vi "Measurement Logic.vi"() -> ()   [LabVIEW 2021, in "Load Transient Response_PMIC.lvlib"]
uses:
  Load Transient Response_PMIC.lvlib
  Measurement Configuration.ctl
  Measurement Results.ctl
  <vilib>/Plug-In SDKs/Measurements/Measure Call Context/Measure Call Context.lvclass
  <instrlib>/niDCPower/nidcpower.llb/niDCPower Sense.ctl
  <instrlib>/niDCPower/nidcpower.llb/niDCPower Source Mode.ctl
  <instrlib>/niDCPower/nidcpower.llb/niDCPower Wait For Event - Event.ctl
  <instrlib>/niDCPower/nidcpower.llb/niDCPower Output Function.ctl
  <instrlib>/niDCPower/nidcpower.llb/niDCPower Aperture Time Units.ctl
  <instrlib>/niDCPower/nidcpower.llb/niDCPower Configure Digital Edge Measure Trigger With Channels.vi
panel:
  out "measure call context out":refnum<class "Measure Call Context.lvclass">
  in  "measure call context in":refnum<class "Measure Call Context.lvclass">
  out "measurement results":T1
  in  "measurement configuration":T2={"Mode of operation"=enum."Perform measurement", "DUT setup time"=1.0, "Nominal output voltage"=3.3, "Source resource name"="", "Source sense"=1009, "Source current limit"=25.0, "Source voltage level"=12.0, "Source transient response"=1041, "Source voltage gain bandwidth"=2000.0, "Source voltage compensation frequency"=3530.0, "Source voltage pole-zero ratio"=2.0, "Load resource name"="", "Load sense"=1009, "Load voltage limit range"=6.0, "Load current level range"=6.0, "Load sample rate"=1800000.0, "Load current set point 1"=1.0, "Load current set point 2"=22.0, "Load current delay t1"=0.001, "Load current pulse duration"=0.001, "Load current delay t2"=0.001, "Load current rising slew rate"=24.0, "Load current falling slew rate"=24.0, "Load transient response"=3, "Load current gain bandwidth"=14000.0, "Load current compensation frequency"=180000.0, "Load current pole-zero ratio"=0.3} {"Load transient response" items=["Slow"=1041, "Normal"=1038, "Fast"=1039, "Custom"=1042]; "Load current rising slew rate" format="%#_6p"; "Load sense" items=["Local"=1008, "Remote"=1009]; "Source transient response" items=["Slow"=1041, "Normal"=1038, "Fast"=1039, "Custom"=1042]; "Source sense" items=["Local"=1008, "Remote"=1009]; "Nominal output voltage" format="%#_6p"}
  out "error out":errorcluster
  in  "error in":errorcluster
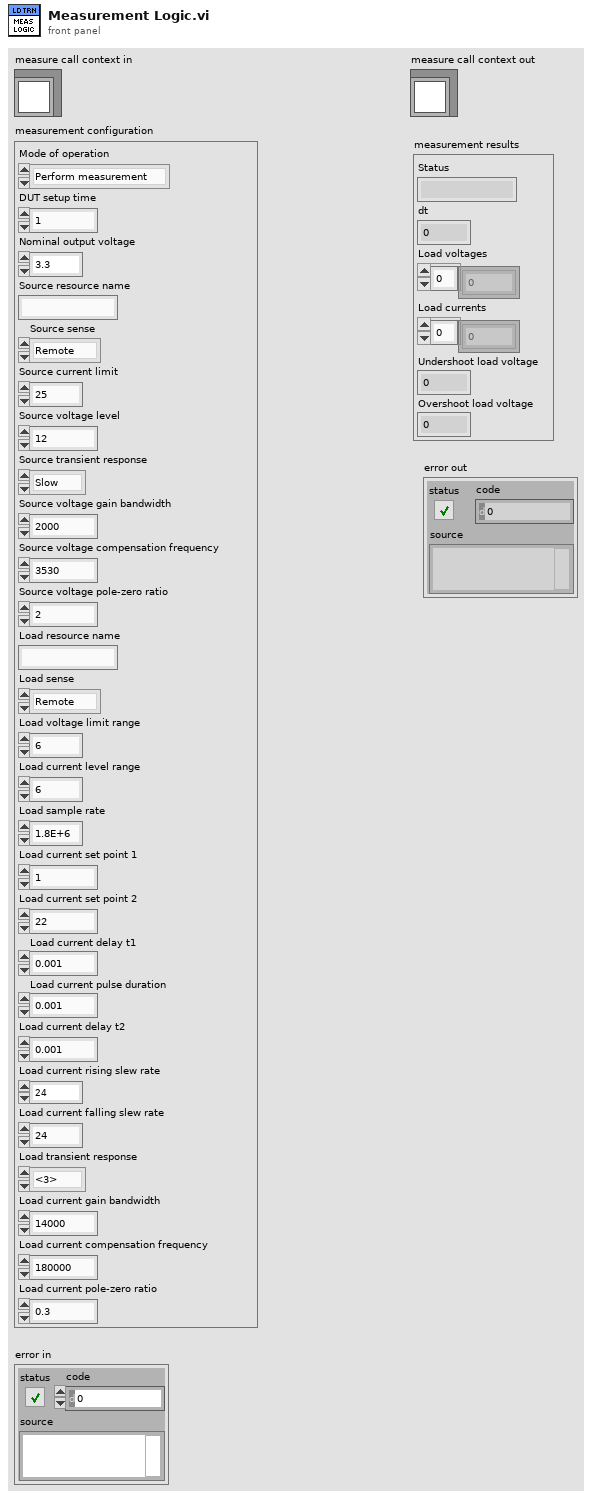
[diagram p1: front panel]
types:
  T1 = typedef "Load Transient Response_PMIC.lvlib/Measurement Results.ctl" = cluster{"Status":string, "dt":dbl, "Load voltages":dbl[], "Load currents":dbl[], "Undershoot load voltage":dbl, "Overshoot load voltage":dbl}
  T2 = typedef "Load Transient Response_PMIC.lvlib/Measurement Configuration.ctl" = cluster{"Mode of operation":enum32{"Power on the DUT", "Perform measurement", "Power off the DUT"}, "DUT setup time":dbl, "Nominal output voltage":dbl, "Source resource name":string, "Source sense":i32, "Source current limit":dbl, "Source voltage level":dbl, "Source transient response":i32, "Source voltage gain bandwidth":dbl, "Source voltage compensation frequency":dbl, "Source voltage pole-zero ratio":dbl, "Load resource name":string, "Load sense":i32, "Load voltage limit range":dbl, "Load current level range":dbl, "Load sample rate":dbl, "Load current set point 1":dbl, "Load current set point 2":dbl, "Load current delay t1":dbl, "Load current pulse duration":dbl, "Load current delay t2":dbl, "Load current rising slew rate":dbl, "Load current falling slew rate":dbl, "Load transient response":i32, "Load current gain bandwidth":dbl, "Load current compensation frequency":dbl, "Load current pole-zero ratio":dbl}
  T3 = cluster{"Source out":refnum<k15>, "Source channel name":string, "Load out":refnum<k15>, "Load channel name":string, "No of samples to fetch":i32, "Measurement Results":T1, "Source voltage level":dbl, "Source current limit":dbl, "Measure terminal name":string, "Loadmodelname":string}
  T4 = enum32{"Power on the DUT", "Perform measurement", "Power off the DUT"}
  T5 = typedef "niDCPower Wait For Event - Event.ctl" = i32
  T6 = typedef "niDCPower Source Mode.ctl" = i32
  T7 = typedef "niDCPower Sense.ctl" = i32
  T8 = typedef "niDCPower Output Function.ctl" = i32
  T9 = typedef "niDCPower Aperture Time Units.ctl" = i32
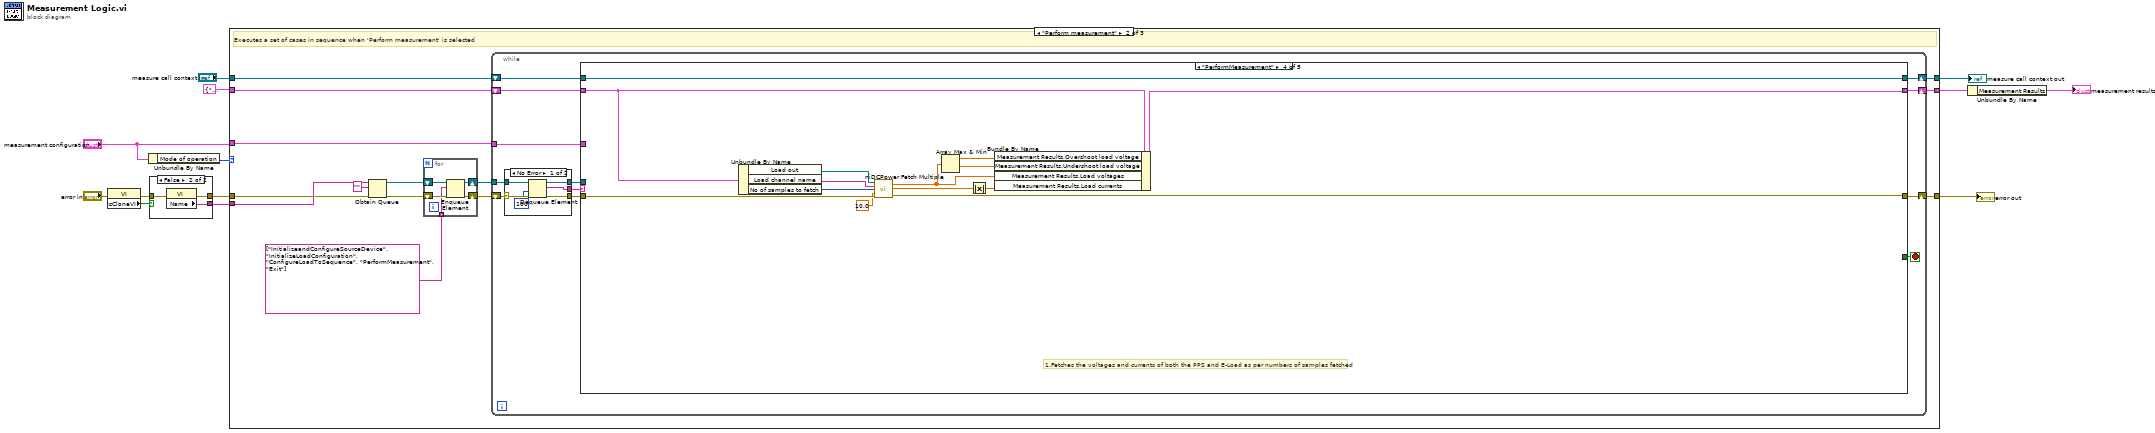
[diagram p0: block diagram]
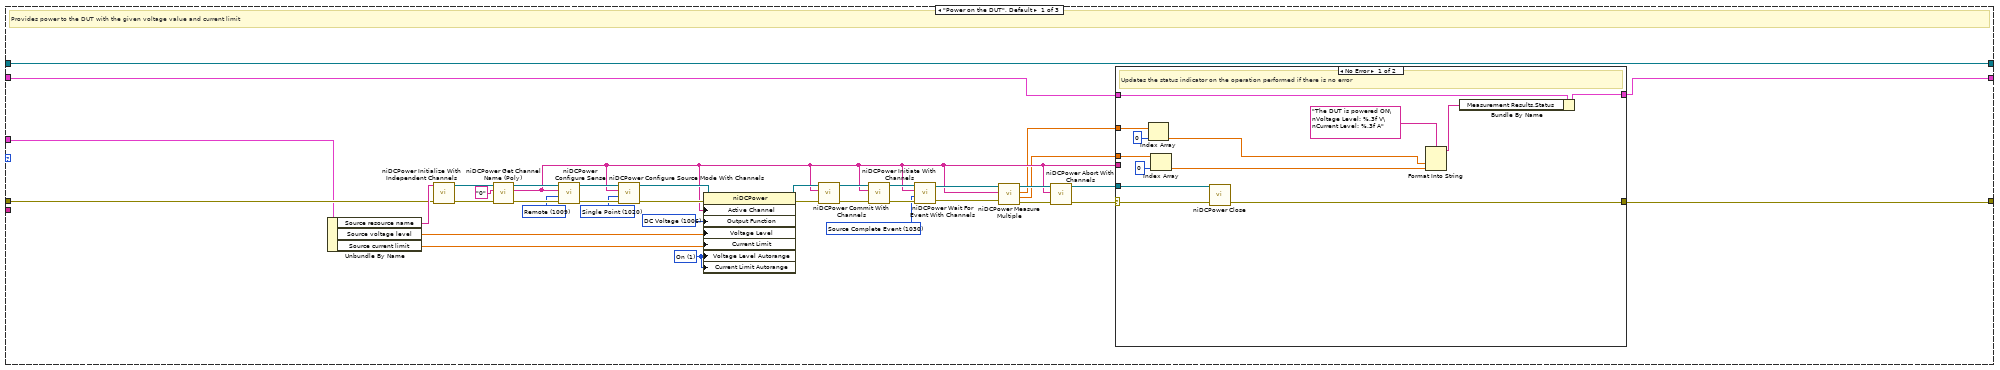
[diagram p2: hidden frame]
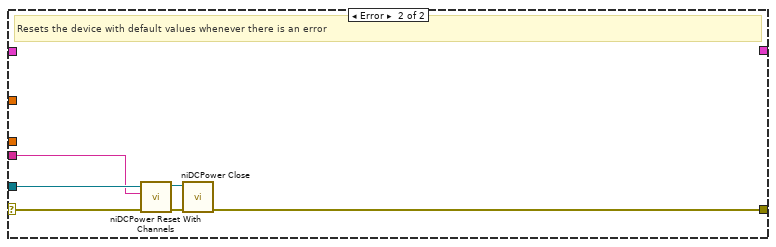
[diagram p3: hidden frame]
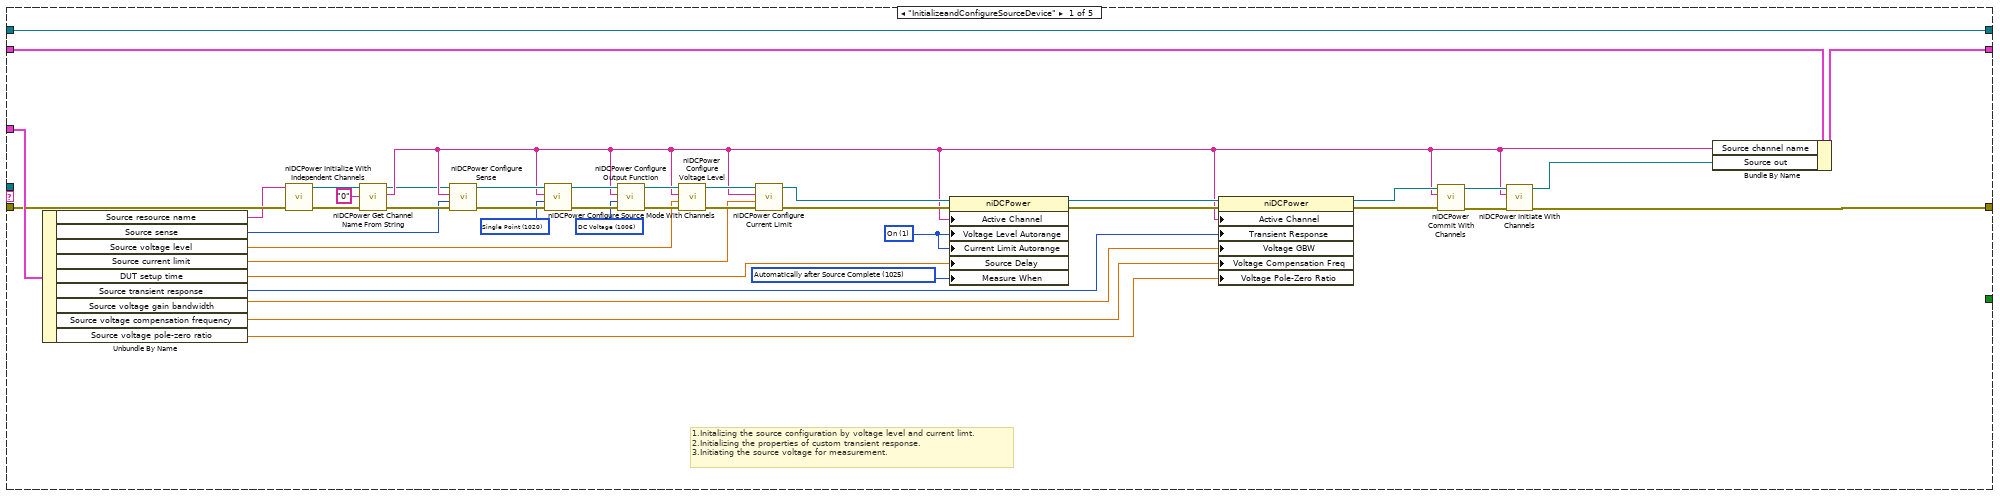
[diagram p4: hidden frame]
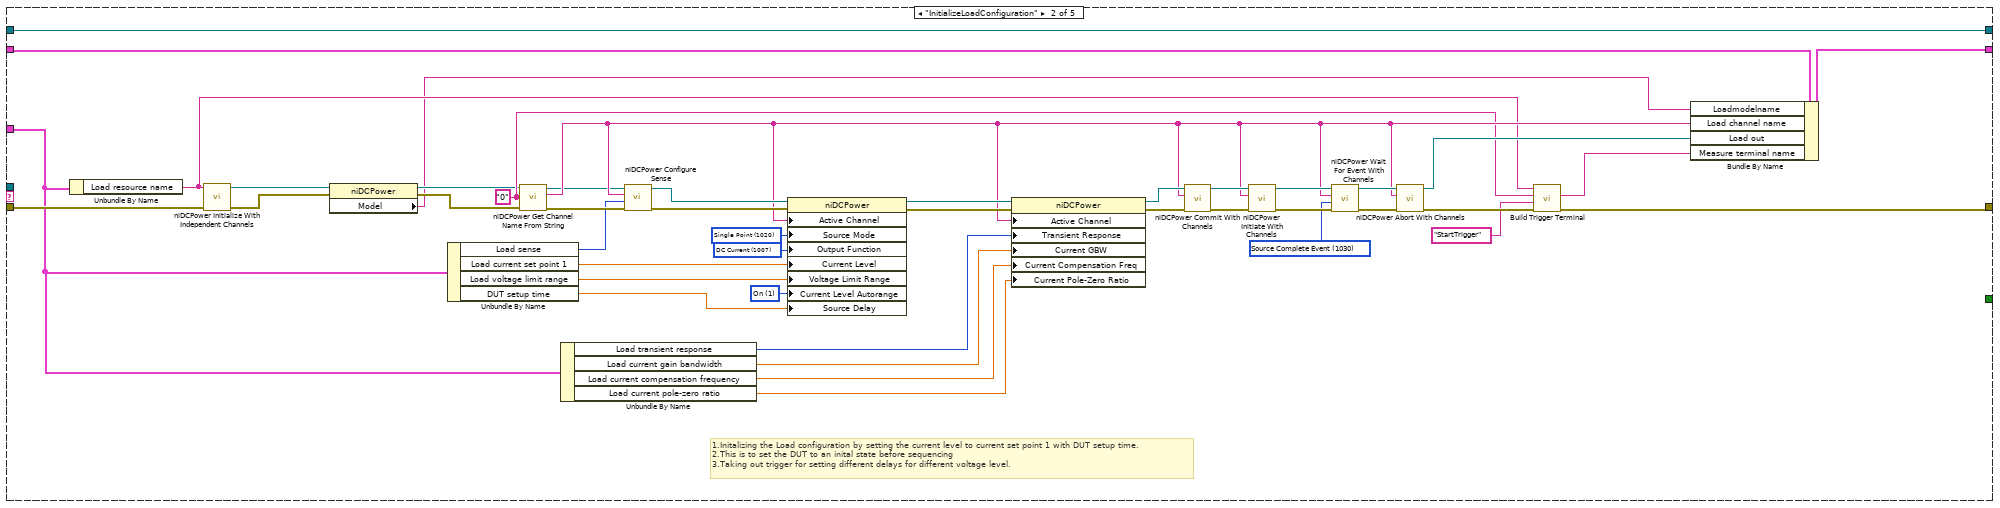
[diagram p5: hidden frame]
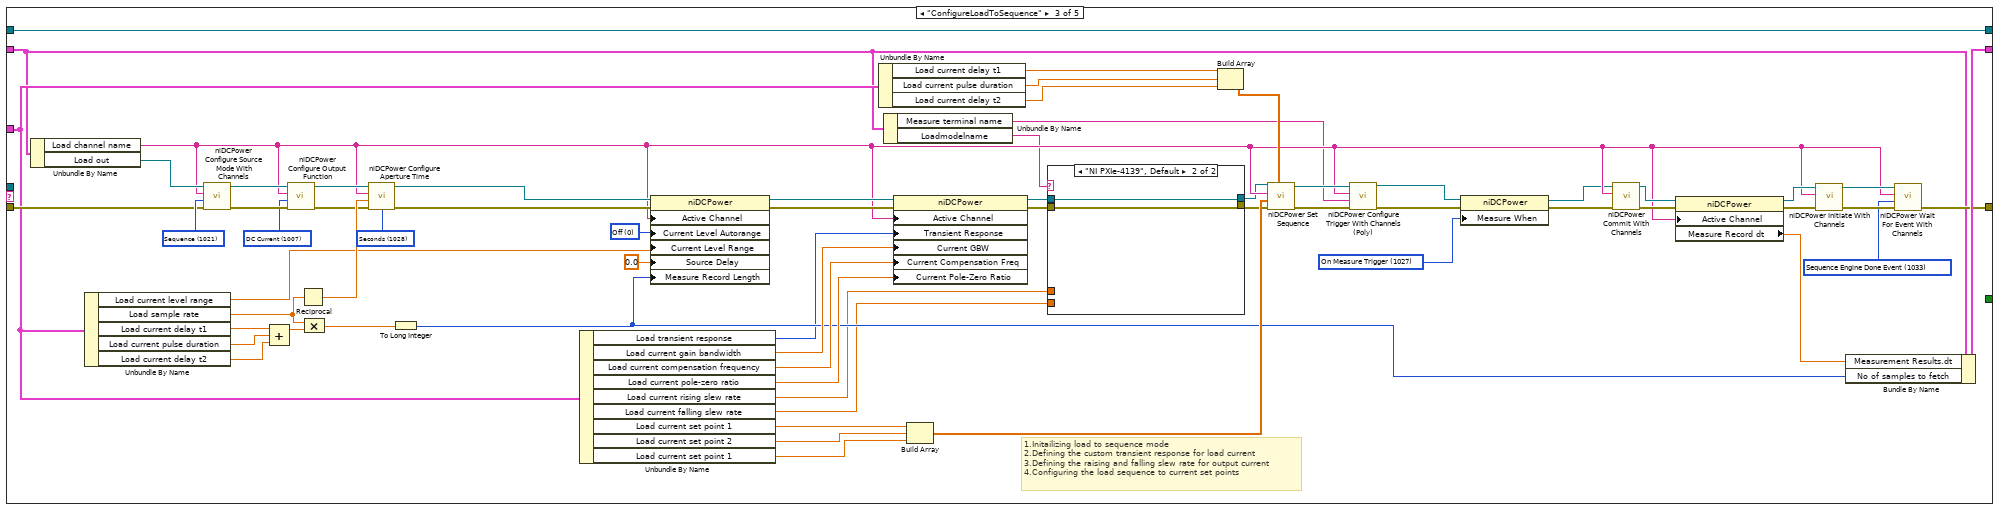
[diagram p6: hidden frame]
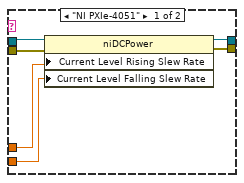
[diagram p7: hidden frame]
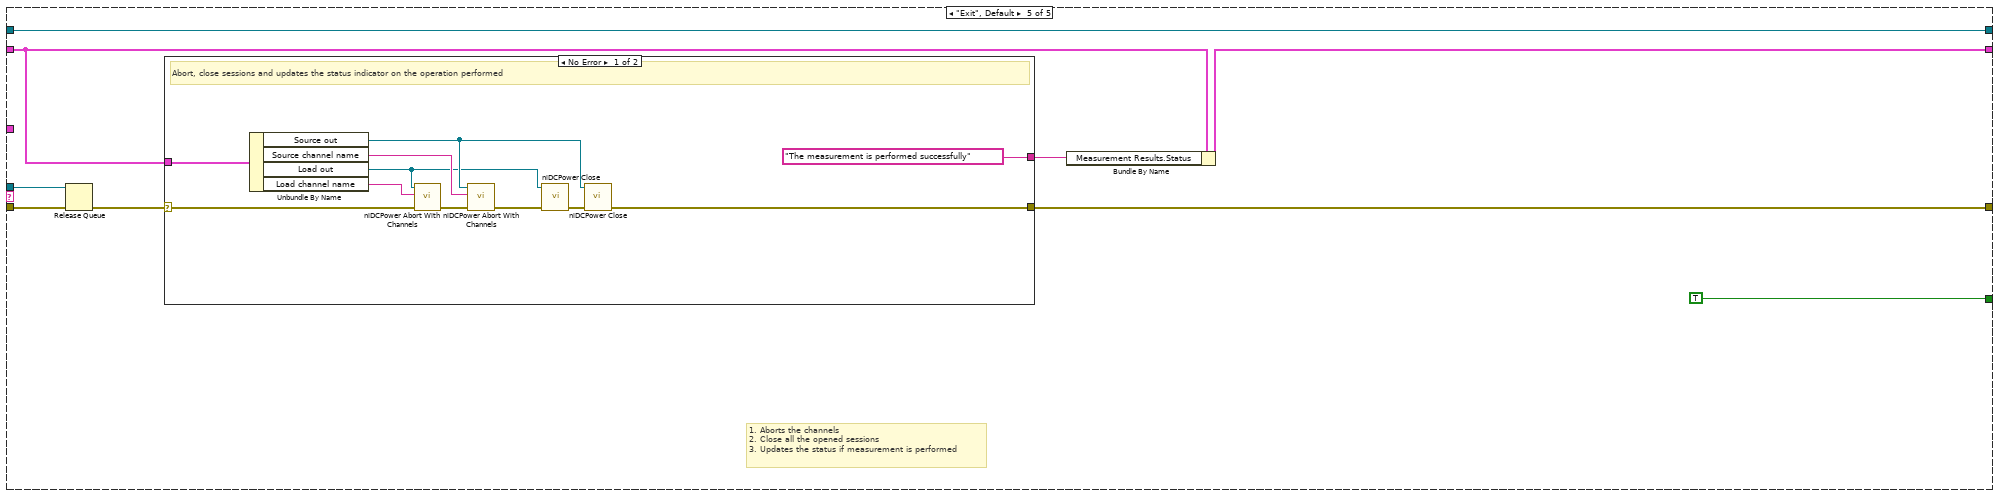
[diagram p8: hidden frame]
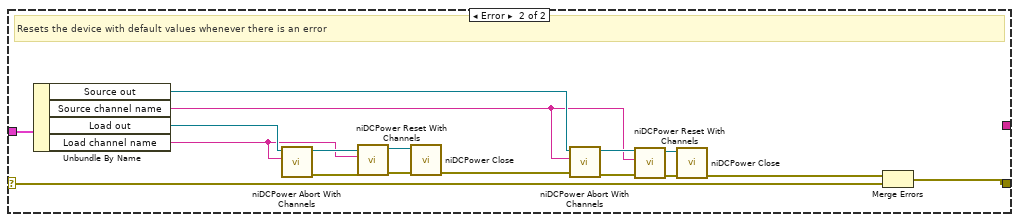
[diagram p9: hidden frame]
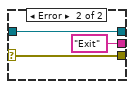
[diagram p10: hidden frame]
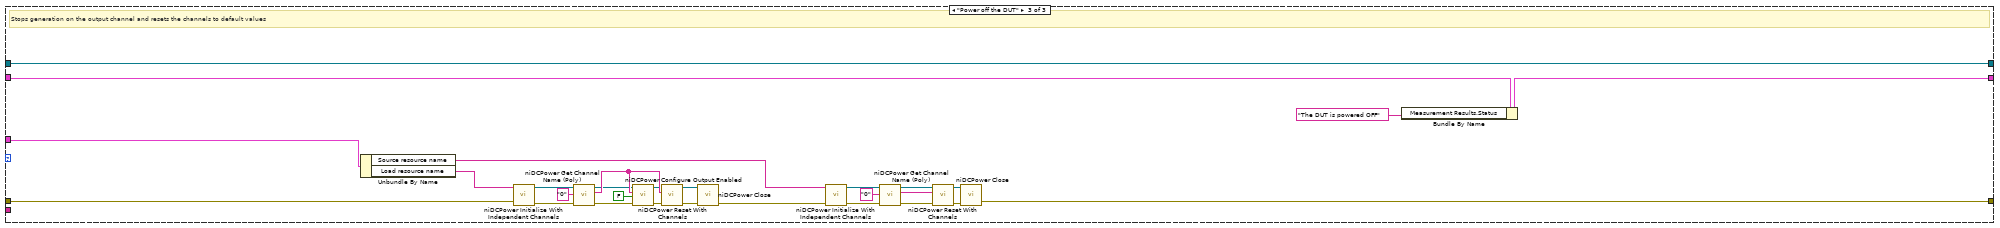
[diagram p11: hidden frame]
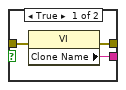
[diagram p12: hidden frame]
diagram:
  n1 = property class="VI"(error in="error in") -> (error out=w12:errorcluster, "IsCloneVI"=w13:bool)  [unwired: 1 in, 1 out]
  n2 = Unbundle By Name("measurement configuration") -> ("Mode of operation"=w2:T4)
  n3 = case shown="False" w13 {
    tunnel: [w16 w19] -> w4
    tunnel: [w15 w18] -> w1
    tunnel: w12 -> [w14 w17]
    frame True {
      n4 = property class="VI"(error in=w14) -> (error out=w16:errorcluster, "Clone Name"=w15:string)  [unwired: 1 in, 1 out]
    }
    frame False {
      n5 = property class="VI"(error in=w17) -> (error out=w19:errorcluster, "Name"=w18:string)  [unwired: 1 in, 1 out]
    }
  }
  n6 = case shown="\"Perform measurement\"" w2 {
    tunnel: T3 {"Source out"="", "Source channel name"="", "Load out"="", "Load channel name"="", "No of samples to fetch"=1, "Measurement Results"={"Status"="", "dt"=0.0, "Load voltages"=[], "Load currents"=[], "Undershoot load voltage"=0.0, "Overshoot load voltage"=0.0}, "Source voltage level"=0.0, "Source current limit"=0.0, "Measure terminal name"="", "Loadmodelname"=""} -> [w30 w89 w329]
    tunnel: "measure call context in" -> [w29 w88 w326]
    tunnel: [w21 w87 w330] -> w8
    tunnel: [w29 w86 w326] -> w6
    tunnel: [w20 w85 w327] -> w5
    tunnel: "measurement configuration" -> [w33 w84 w332]
    tunnel: w4 -> [w34 w77 w331]
    tunnel: w1 -> [_ w80 _]
    frame "Power on the DUT", Default {
      w38 = 1 items=["Off", "On"] ("Source:DC Voltage:Voltage Level Autorange")
      w37 = T5 1030 items=["Source Complete Event"=1030, "Measure Complete Event"=1031, "Sequence Iteration Complete Event"=1032, "Sequence Engine Done Event"=1033, "Pulse Complete Event"=1051, "Ready For Pulse Trigger Event"=1052] ("event")
      w36 = T6 1020 items=["Single Point"=1020, "Sequence"=1021] ("source mode")
      w39 = 1006 items=["DC Voltage"=1006, "DC Current"=1007, "Pulse Voltage"=1049, "Pulse Current"=1050] ("Source:Output Function")
      w40 = T7 1009 items=["Local"=1008, "Remote"=1009] ("sense")
      # "Provides power to the DUT with the given voltage value and current limit"
      n7 = Unbundle By Name(w33) -> ("Source resource name"=w54:string, "Source voltage level"=w55:dbl, "Source current limit"=w56:dbl)
      n8 = call <instrlib>:"niDCPower Initialize With Independent Channels.vi"("error in (no error)"=w34, "resource name"=w54) -> ("error out"=w52:errorcluster, "instrument handle out"=w51:refnum<k15>)  [unwired: 8 in]
      n9 = call-poly <instrlib>:"niDCPower Get Channel Name (Poly).vi"("index"="0", "instrument handle"=w51) -> ("name"=w26:string, "instrument handle out"=w53:refnum<k15>)  [unwired: 7 in, 1 out]
      n10 = call <instrlib>:"niDCPower Configure Sense.vi"("error in (no error)"=w52, "sense"=w40, "channel name"=w26, "instrument handle"=w53) -> ("error out"=w46:errorcluster, "instrument handle out"=w48:refnum<k15>)  [unwired: 6 in]
      n11 = call <instrlib>:"niDCPower Configure Source Mode With Channels.vi"("error in (no error)"=w46, "source mode"=w36, "channel name"=w26, "instrument handle"=w48) -> ("error out"=w45:errorcluster, "instrument handle out"=w47:refnum<k15>)  [unwired: 6 in]
      n12 = property class="niDCPower"(reference=w47, error in=w45, "Active Channel"=w26, "Output Function"=w39, "Voltage Level"=w55, "Current Limit"=w56, "Voltage Level Autorange"=w38, "Current Limit Autorange"=w38) -> (reference out=w44:refnum<k15>, error out=w43:errorcluster)
      n13 = call <instrlib>:"niDCPower Commit With Channels.vi"("error in (no error)"=w43, "channel name"=w26, "instrument handle"=w44) -> ("error out"=w41:errorcluster, "instrument handle out"=w42:refnum<k15>)  [unwired: 7 in]
      n14 = call <instrlib>:"niDCPower Initiate With Channels.vi"("error in (no error)"=w41, "channel name"=w26, "instrument handle"=w42) -> ("error out"=w50:errorcluster, "instrument handle out"=w49:refnum<k15>)  [unwired: 7 in]
      n15 = call <instrlib>:"niDCPower Wait For Event With Channels.vi"("error in (no error)"=w50, "event"=w37, "channel name"=w26, "instrument handle"=w49) -> ("error out"=w25:errorcluster, "instrument handle out"=w28:refnum<k15>)  [unwired: 6 in]
      n16 = call <instrlib>:"niDCPower Measure Multiple.vi"("error in (no error)"=w25, "channel name"=w26, "instrument handle"=w28) -> ("error out"=w24:errorcluster, "current measurements"=w22:dbl[], "voltage measurements"=w23:dbl[], "instrument handle out"=w27:refnum<k15>)  [unwired: 5 in]
      n17 = call <instrlib>:"niDCPower Abort With Channels.vi"("error in (no error)"=w24, "channel name"=w26, "instrument handle"=w27) -> ("error out"=w32:errorcluster, "instrument handle out"=w31:refnum<k15>)  [unwired: 7 in]
      n18 = case shown="No Error" w32 {
        selector: w32 -> [w68 w72]
        tunnel: [w67 w71] -> w21
        tunnel: w31 -> [w69 w73]
        tunnel: w26 -> [_ w70]
        tunnel: w30 -> [w66 _]
        tunnel: [w65 _] -> w20
        tunnel: w23 -> [w62 _]
        tunnel: w22 -> [w61 _]
        frame No Error {
          # "Updates the status indicator on the operation performed if there is no error"
          n19 = Index Array(array=w62, index=0) -> (element=w58:dbl)
          n20 = Index Array(array=w61, index=0) -> (element=w57:dbl)
          n21 = call <instrlib>:"niDCPower Close.vi"("error in (no error)"=w68, "instrument handle"=w69) -> ("error out"=w67:errorcluster)  [unwired: 9 out]
          n22 = Format Into String(format string="The DUT is powered ON\nVoltage Level: %.3f V\nCurrent Level: %.3f A" ("message"), w58, w57) -> (resulting string=w63:string)  [unwired: 2 in, 1 out]
          n23 = Bundle By Name(cluster=w66, "Measurement Results.Status"=w63) -> (w65:T3)
        }
        frame Error {
          # "Resets the device with default values whenever there is an error"
          n24 = call <instrlib>:"niDCPower Reset With Channels.vi"("error in (no error)"=w72, "channel name"=w70, "instrument handle"=w73) -> ("error out"=w75:errorcluster, "instrument handle out"=w74:refnum<k15>)  [unwired: 7 in]
          n25 = call <instrlib>:"niDCPower Close.vi"("error in (no error)"=w75, "instrument handle"=w74) -> ("error out"=w71:errorcluster)  [unwired: 9 out]
        }
      }
    }
    frame "Perform measurement" {
      # "Executes a set of cases in sequence when 'Perform measurement' is selected"
      n26 = Obtain Queue(name (unnamed)=w80, element data type="", error in (no error)=w77) -> (queue out=w79:refnum<queue>, error out=w78:errorcluster)  [unwired: 2 in, 1 out]
      n27 = for {
        tunnel: string[] ["InitializeandConfigureSourceDevice", "InitializeLoadConfiguration", "ConfigureLoadToSequence", "PerformMeasurement", "Exit"] ("Step sequence") -> [w90] mode=indexing
        shift-right: [w93] -> w81
        shift-left: w79 -> [w92]
        shift-right: [w94] -> w82
        shift-left: w78 -> [w91]
        n28 = Enqueue Element(queue=w92, element=w90, error in (no error)=w91) -> (queue out=w93:refnum<queue>, error out=w94:errorcluster)  [unwired: 1 in, 1 out]
      }
      n29 = while {
        tunnel: w81 -> [w106]
        shift-right: [w99] -> w87
        shift-left: w82 -> [w105]
        tunnel: w84 -> [w101]
        shift-right: [w96] -> w86
        shift-left: w88 -> [w97]
        shift-right: [w95] -> w85
        shift-left: w89 -> [w98]
        stop <- w100 stop-if-true
        n30 = case shown="No Error" w105 {
          selector: w105 -> [w320 w324]
          tunnel: w106 -> [w322 w323]
          tunnel: [w321 "Exit" ("t")] -> w104
          tunnel: [w319 w324] -> w102
          tunnel: [w317 w323] -> w103
          frame No Error {
            n31 = Dequeue Element(queue=w322, timeout in ms (-1)=100, error in (no error)=w320) -> (queue out=w317:refnum<queue>, element=w321:string, error out=w319:errorcluster)  [unwired: 1 out]
          }
          frame Error {
          }
        }
        n32 = case shown="\"PerformMeasurement\"" w104 {
          tunnel: w103 -> [_ _ _ _ w286]
          tunnel: w102 -> [w127 w178 w231 w277 w285]
          tunnel: w101 -> [w134 w177 w214 _ _]
          tunnel: [_ _ _ _ TRUE] -> w100
          tunnel: [w110 w159 w224 w275 w280] -> w99
          tunnel: w98 -> [w125 w172 w206 w278 w283]
          tunnel: w97 -> [w126 w169 w225 w279 w287]
          tunnel: [w126 w169 w225 w279 w287] -> w96
          tunnel: [w123 w170 w230 w276 w282] -> w95
          frame "InitializeandConfigureSourceDevice" {
            w129 = 1025 items=["Automatically after Source Complete"=1025, "On Demand"=1026, "On Measure Trigger"=1027] ("Measurement:Advanced:Measure When")
            w135 = 1 items=["Off", "On"] ("Source:DC Voltage:Current Limit Autorange")
            w136 = T8 1006 items=["DC Voltage"=1006, "DC Current"=1007, "Pulse Voltage"=1049, "Pulse Current"=1050] ("output function")
            w137 = T6 1020 items=["Single Point"=1020, "Sequence"=1021] ("source mode")
            # "1.Initalizing the source configuration by voltage level and current limt.\n2.Initializing the properties of custom transient response.\n3.Initiating the source voltage for measurement."
            n33 = Unbundle By Name(w134) -> ("Source resource name"=w109:string, "Source sense"=w108:i32, "Source voltage level"=w113:dbl, "Source current limit"=w114:dbl, "DUT setup time"=w115:dbl, "Source transient response"=w112:i32, "Source voltage gain bandwidth"=w128:dbl, "Source voltage compensation frequency"=w122:dbl, "Source voltage pole-zero ratio"=w107:dbl)
            n34 = call <instrlib>:"niDCPower Initialize With Independent Channels.vi"("error in (no error)"=w127, "resource name"=w109) -> ("error out"=w117:errorcluster, "instrument handle out"=w120:refnum<k15>)  [unwired: 8 in]
            n35 = call <instrlib>:"niDCPower Get Channel Name From String.vi"("error in (no error)"=w117, "index"="0", "instrument handle"=w120) -> ("error out"=w116:errorcluster, "name"=w119:string, "instrument handle out"=w118:refnum<k15>)  [unwired: 6 in]
            n36 = call <instrlib>:"niDCPower Configure Sense.vi"("error in (no error)"=w116, "sense"=w108, "channel name"=w119, "instrument handle"=w118) -> ("error out"=w147:errorcluster, "instrument handle out"=w148:refnum<k15>)  [unwired: 6 in]
            n37 = call <instrlib>:"niDCPower Configure Source Mode With Channels.vi"("error in (no error)"=w147, "source mode"=w137, "channel name"=w119, "instrument handle"=w148) -> ("error out"=w138:errorcluster, "instrument handle out"=w139:refnum<k15>)  [unwired: 6 in]
            n38 = call <instrlib>:"niDCPower Configure Output Function.vi"("error in (no error)"=w138, "output function"=w136, "channel name"=w119, "instrument handle"=w139) -> ("error out"=w141:errorcluster, "instrument handle out"=w142:refnum<k15>)  [unwired: 6 in]
            n39 = call <instrlib>:"niDCPower Configure Voltage Level.vi"("error in (no error)"=w141, "voltage level"=w113, "channel name"=w119, "instrument handle"=w142) -> ("error out"=w144:errorcluster, "instrument handle out"=w143:refnum<k15>)  [unwired: 6 in]
            n40 = call <instrlib>:"niDCPower Configure Current Limit.vi"("error in (no error)"=w144, "current limit"=w114, "channel name"=w119, "instrument handle"=w143) -> ("error out"=w140:errorcluster, "instrument handle out"=w121:refnum<k15>)  [unwired: 6 in]
            n41 = property class="niDCPower"(reference=w121, error in=w140, "Active Channel"=w119, "Voltage Level Autorange"=w135, "Current Limit Autorange"=w135, "Source Delay"=w115, "Measure When"=w129) -> (reference out=w133:refnum<k15>, error out=w131:errorcluster)
            n42 = property class="niDCPower"(reference=w133, error in=w131, "Active Channel"=w119, "Transient Response"=w112, "Voltage GBW"=w128, "Voltage Compensation Freq"=w122, "Voltage Pole-Zero Ratio"=w107) -> (reference out=w132:refnum<k15>, error out=w130:errorcluster)
            n43 = call <instrlib>:"niDCPower Commit With Channels.vi"("error in (no error)"=w130, "channel name"=w119, "instrument handle"=w132) -> ("error out"=w146:errorcluster, "instrument handle out"=w145:refnum<k15>)  [unwired: 7 in]
            n44 = call <instrlib>:"niDCPower Initiate With Channels.vi"("error in (no error)"=w146, "channel name"=w119, "instrument handle"=w145) -> ("error out"=w110:errorcluster, "instrument handle out"=w124:refnum<k15>)  [unwired: 7 in]
            n45 = Bundle By Name(cluster=w125, "Source channel name"=w119, "Source out"=w124) -> (w123:T3)
          }
          frame "InitializeLoadConfiguration" {
            w157 = "0" ("index")
            w179 = 1 items=["Off", "On"] ("Source:DC Current:Current Level Autorange")
            w188 = T5 1030 items=["Source Complete Event"=1030, "Measure Complete Event"=1031, "Sequence Iteration Complete Event"=1032, "Sequence Engine Done Event"=1033, "Pulse Complete Event"=1051, "Ready For Pulse Trigger Event"=1052] ("event")
            w191 = 1007 items=["DC Voltage"=1006, "DC Current"=1007, "Pulse Voltage"=1049, "Pulse Current"=1050] ("Source:Output Function")
            w192 = 1020 items=["Single Point"=1020, "Sequence"=1021] ("Source:Source Mode")
            # "1.Initalizing the Load configuration by setting the current level to current set point 1 with DUT setup time.\n2.This is to set the DUT to an inital state before sequencing\n3.Taking out trigger for setting different delays for different voltage level."
            n46 = Unbundle By Name(w177) -> ("Load resource name"=w158:string)
            n47 = call <instrlib>:"niDCPower Initialize With Independent Channels.vi"("error in (no error)"=w178, "resource name"=w158) -> ("error out"=w151:errorcluster, "instrument handle out"=w153:refnum<k15>)  [unwired: 8 in]
            n48 = property class="niDCPower"(reference=w153, error in=w151) -> (reference out=w152:refnum<k15>, error out=w150:errorcluster, "Model"=w149:string)
            n49 = Unbundle By Name(w177) -> ("Load sense"=w154:i32, "Load current set point 1"=w167:dbl, "Load voltage limit range"=w168:dbl, "DUT setup time"=w176:dbl)
            n50 = call <instrlib>:"niDCPower Get Channel Name From String.vi"("error in (no error)"=w150, "index"=w157, "instrument handle"=w152) -> ("error out"=w162:errorcluster, "name"=w164:string, "instrument handle out"=w163:refnum<k15>)  [unwired: 6 in]
            n51 = Unbundle By Name(w177) -> ("Load transient response"=w161:i32, "Load current gain bandwidth"=w175:dbl, "Load current compensation frequency"=w174:dbl, "Load current pole-zero ratio"=w173:dbl)
            n52 = call <instrlib>:"niDCPower Configure Sense.vi"("error in (no error)"=w162, "sense"=w154, "channel name"=w164, "instrument handle"=w163) -> ("error out"=w184:errorcluster, "instrument handle out"=w185:refnum<k15>)  [unwired: 6 in]
            n53 = property class="niDCPower"(reference=w185, error in=w184, "Active Channel"=w164, "Source Mode"=w192, "Output Function"=w191, "Current Level"=w167, "Voltage Limit Range"=w168, "Current Level Autorange"=w179, "Source Delay"=w176) -> (reference out=w181:refnum<k15>, error out=w180:errorcluster)
            n54 = property class="niDCPower"(reference=w181, error in=w180, "Active Channel"=w164, "Transient Response"=w161, "Current GBW"=w175, "Current Compensation Freq"=w174, "Current Pole-Zero Ratio"=w173) -> (reference out=w166:refnum<k15>, error out=w165:errorcluster)
            n55 = call <instrlib>:"niDCPower Commit With Channels.vi"("error in (no error)"=w165, "channel name"=w164, "instrument handle"=w166) -> ("error out"=w182:errorcluster, "instrument handle out"=w183:refnum<k15>)  [unwired: 7 in]
            n56 = call <instrlib>:"niDCPower Initiate With Channels.vi"("error in (no error)"=w182, "channel name"=w164, "instrument handle"=w183) -> ("error out"=w190:errorcluster, "instrument handle out"=w189:refnum<k15>)  [unwired: 7 in]
            n57 = call <instrlib>:"niDCPower Wait For Event With Channels.vi"("error in (no error)"=w190, "event"=w188, "channel name"=w164, "instrument handle"=w189) -> ("error out"=w187:errorcluster, "instrument handle out"=w186:refnum<k15>)  [unwired: 6 in]
            n58 = call <instrlib>:"niDCPower Abort With Channels.vi"("error in (no error)"=w187, "channel name"=w164, "instrument handle"=w186) -> ("error out"=w160:errorcluster, "instrument handle out"=w171:refnum<k15>)  [unwired: 7 in]
            n59 = call "Build Trigger Terminal.vi"("error in (no error)"=w160, "Trigger/Event Name"="StartTrigger" ("Trigger Type"), "Channel Name"=w157, "Resource Name"=w158) -> ("error out"=w159:errorcluster, "Terminal Name"=w156:string)  [unwired: 6 in]
            n60 = Bundle By Name(cluster=w172, "Loadmodelname"=w149, "Load channel name"=w164, "Load out"=w171, "Measure terminal name"=w156) -> (w170:T3)
          }
          frame "ConfigureLoadToSequence" {
            w204 = 1027 items=["Automatically after Source Complete"=1025, "On Demand"=1026, "On Measure Trigger"=1027] ("Measurement:Advanced:Measure When")
            w220 = 0 items=["Off", "On"] ("Source:DC Current:Current Level Autorange")
            w240 = T9 1028 items=["Seconds"=1028, "Powerline Cycles"=1029] ("aperture time units")
            w239 = T8 1007 items=["DC Voltage"=1006, "DC Current"=1007, "Pulse Voltage"=1049, "Pulse Current"=1050] ("output function")
            w241 = T5 1033 items=["Source Complete Event"=1030, "Measure Complete Event"=1031, "Sequence Iteration Complete Event"=1032, "Sequence Engine Done Event"=1033, "Pulse Complete Event"=1051, "Ready For Pulse Trigger Event"=1052] ("event")
            w242 = T6 1021 items=["Single Point"=1020, "Sequence"=1021] ("source mode")
            # "1.Initailizing load to sequence mode\n2.Defining the custom transient response for load current\n3.Defining the raising and falling slew rate for output current\n4.Configuring the load sequence to current set points"
            n61 = Unbundle By Name(w206) -> ("Load channel name"=w208:string, "Load out"=w235:refnum<k15>)
            n62 = Unbundle By Name(w214) -> ("Load current level range"=w219:dbl, "Load sample rate"=w254:dbl, "Load current delay t1"=w217:dbl, "Load current pulse duration"=w216:dbl, "Load current delay t2"=w215:dbl)
            n63 = call <instrlib>:"niDCPower Configure Source Mode With Channels.vi"("error in (no error)"=w231, "source mode"=w242, "channel name"=w208, "instrument handle"=w235) -> ("error out"=w246:errorcluster, "instrument handle out"=w245:refnum<k15>)  [unwired: 6 in]
            n64 = Compound Arithmetic op=ADD(w217, w216, w215) -> (w218:dbl)
            n65 = call <instrlib>:"niDCPower Configure Output Function.vi"("error in (no error)"=w246, "output function"=w239, "channel name"=w208, "instrument handle"=w245) -> ("error out"=w248:errorcluster, "instrument handle out"=w247:refnum<k15>)  [unwired: 6 in]
            n66 = Reciprocal(x=w254) -> (1/x=w249:dbl)
            n67 = Compound Arithmetic op=MULTIPLY(w254, w218) -> (w251:dbl)
            n68 = call <instrlib>:"niDCPower Configure Aperture Time.vi"("aperture time units"=w240, "error in (no error)"=w248, "aperture time"=w249, "channel name"=w208, "instrument handle"=w247) -> ("error out"=w237:errorcluster, "instrument handle out"=w236:refnum<k15>)  [unwired: 5 in]
            n69 = To Long Integer(number=w251) -> (32bit integer=w222:i32)
            n70 = Unbundle By Name(w214) -> ("Load transient response"=w221:i32, "Load current gain bandwidth"=w234:dbl, "Load current compensation frequency"=w233:dbl, "Load current pole-zero ratio"=w232:dbl, "Load current rising slew rate"=w194:dbl, "Load current falling slew rate"=w193:dbl, "Load current set point 1"=w229:dbl, "Load current set point 2"=w228:dbl, "Load current set point 1"=w227:dbl)
            n71 = property class="niDCPower"(reference=w236, error in=w237, "Active Channel"=w208, "Current Level Autorange"=w220, "Current Level Range"=w219, "Source Delay"=0.0 ("Source:Advanced:Source Delay"), "Measure Record Length"=w222) -> (reference out=w256:refnum<k15>, error out=w257:errorcluster)
            n72 = Unbundle By Name(w214) -> ("Load current delay t1"=w213:dbl, "Load current pulse duration"=w212:dbl, "Load current delay t2"=w211:dbl)
            n73 = Unbundle By Name(w206) -> ("Measure terminal name"=w205:string, "Loadmodelname"=w199:string)
            n74 = property class="niDCPower"(reference=w256, error in=w257, "Active Channel"=w208, "Transient Response"=w221, "Current GBW"=w234, "Current Compensation Freq"=w233, "Current Pole-Zero Ratio"=w232) -> (reference out=w198:refnum<k15>, error out=w197:errorcluster)
            n75 = Build Array(w229, w228, w227) -> (w226:dbl[])
            n76 = case shown="\"NI PXIe-4139\", Default" w199 {
              tunnel: [w261 w265] -> w195
              tunnel: w198 -> [w263 w265]
              tunnel: [w260 w264] -> w196
              tunnel: w197 -> [w262 w264]
              tunnel: w194 -> [w259 _]
              tunnel: w193 -> [w258 _]
              frame "NI PXIe-4051" {
                n77 = property class="niDCPower"(reference=w263, error in=w262, "Current Level Rising Slew Rate"=w259, "Current Level Falling Slew Rate"=w258) -> (reference out=w261:refnum<k15>, error out=w260:errorcluster)
              }
              frame "NI PXIe-4139", Default {
              }
            }
            n78 = Build Array(w213, w212, w211) -> (w210:dbl[])
            n79 = call <instrlib>:"niDCPower Set Sequence.vi"("source delays"=w210, "error in (no error)"=w196, "values"=w226, "channel name"=w208, "instrument handle"=w195) -> ("error out"=w207:errorcluster, "instrument handle out"=w209:refnum<k15>)  [unwired: 5 in]
            n80 = call-poly <instrlib>:"niDCPower Configure Trigger With Channels (Poly).vi"("error in (no error)"=w207, "input terminal"=w205, "channel name"=w208, "instrument handle"=w209) -> ("error out"=w201:errorcluster, "instrument handle out"=w203:refnum<k15>)  [unwired: 6 in]
            n81 = property class="niDCPower"(reference=w203, error in=w201, "Measure When"=w204) -> (reference out=w202:refnum<k15>, error out=w200:errorcluster)
            n82 = call <instrlib>:"niDCPower Commit With Channels.vi"("error in (no error)"=w200, "channel name"=w208, "instrument handle"=w202) -> ("error out"=w255:errorcluster, "instrument handle out"=w250:refnum<k15>)  [unwired: 7 in]
            n83 = property class="niDCPower"(reference=w250, error in=w255, "Active Channel"=w208) -> (reference out=w244:refnum<k15>, error out=w243:errorcluster, "Measure Record dt"=w223:dbl)
            n84 = call <instrlib>:"niDCPower Initiate With Channels.vi"("error in (no error)"=w243, "channel name"=w208, "instrument handle"=w244) -> ("error out"=w253:errorcluster, "instrument handle out"=w252:refnum<k15>)  [unwired: 7 in]
            n85 = Bundle By Name(cluster=w206, "Measurement Results.dt"=w223, "No of samples to fetch"=w222) -> (w230:T3)
            n86 = call <instrlib>:"niDCPower Wait For Event With Channels.vi"("error in (no error)"=w253, "event"=w241, "channel name"=w208, "instrument handle"=w252) -> ("error out"=w224:errorcluster)  [unwired: 6 in, 1 out]
          }
          frame "PerformMeasurement" {
            # "1.Fetches the voltages and currents of both the PPS and E-Load as per numbers of samples fetched"
            n87 = Unbundle By Name(w278) -> ("Load out"=w274:refnum<k15>, "Load channel name"=w273:string, "No of samples to fetch"=w272:i32)
            n88 = call <instrlib>:"niDCPower Fetch Multiple.vi"("instrument handle"=w274, "channel name"=w273, "count (1)"=w272, "timeout (1.0)"=10.0, "error in (no error)"=w277) -> ("voltage measurements"=w269:dbl[], "current measurements"=w271:dbl[], "error out"=w275:errorcluster)  [unwired: 5 in, 3 out]
            n89 = Array Max & Min(array=w269) -> (max value=w267:dbl, min value=w268:dbl)  [unwired: 2 out]
            n90 = Absolute Value(x=w271) -> (abs(x)=w266:dbl[])
            n91 = Bundle By Name(cluster=w278, "Measurement Results.Overshoot load voltage"=w267, "Measurement Results.Undershoot load voltage"=w268, "Measurement Results.Load voltages"=w269, "Measurement Results.Load currents"=w266) -> (w276:T3)
          }
          frame "Exit", Default {
            # "1. Aborts the channels\n2. Close all the opened sessions\n3. Updates the status if measurement is performed"
            n92 = Release Queue(queue=w286, error in (no error)=w285) -> (error out=w284:errorcluster)  [unwired: 1 in, 2 out]
            n93 = case shown="No Error" w284 {
              selector: w284 -> [w292 w306]
              tunnel: w283 -> [w290 w307]
              tunnel: [w291 w305] -> w280
              tunnel: ["The measurement is performed successfully" ("message") _] -> w281
              frame No Error {
                # "Abort, close sessions and updates the status indicator on the operation performed"
                n94 = Unbundle By Name(w290) -> ("Source out"=w296:refnum<k15>, "Source channel name"=w298:string, "Load out"=w295:refnum<k15>, "Load channel name"=w297:string)
                n95 = call <instrlib>:"niDCPower Abort With Channels.vi"("error in (no error)"=w292, "channel name"=w297, "instrument handle"=w295) -> ("error out"=w299:errorcluster)  [unwired: 7 in, 1 out]
                n96 = call <instrlib>:"niDCPower Abort With Channels.vi"("error in (no error)"=w299, "channel name"=w298, "instrument handle"=w296) -> ("error out"=w294:errorcluster)  [unwired: 7 in, 1 out]
                n97 = call <instrlib>:"niDCPower Close.vi"("error in (no error)"=w294, "instrument handle"=w295) -> ("error out"=w293:errorcluster)  [unwired: 9 out]
                n98 = call <instrlib>:"niDCPower Close.vi"("error in (no error)"=w293, "instrument handle"=w296) -> ("error out"=w291:errorcluster)  [unwired: 9 out]
              }
              frame Error {
                # "Resets the device with default values whenever there is an error"
                n99 = Unbundle By Name(w307) -> ("Source out"=w301:refnum<k15>, "Source channel name"=w300:string, "Load out"=w303:refnum<k15>, "Load channel name"=w302:string)
                n100 = call <instrlib>:"niDCPower Abort With Channels.vi"("channel name"=w302, "instrument handle"=w303) -> ("error out"=w312:errorcluster, "instrument handle out"=w315:refnum<k15>)  [unwired: 8 in]
                n101 = call <instrlib>:"niDCPower Reset With Channels.vi"("error in (no error)"=w312, "channel name"=w302, "instrument handle"=w315) -> ("error out"=w311:errorcluster, "instrument handle out"=w310:refnum<k15>)  [unwired: 7 in]
                n102 = call <instrlib>:"niDCPower Close.vi"("error in (no error)"=w311, "instrument handle"=w310) -> ("error out"=w316:errorcluster)  [unwired: 9 out]
                n103 = call <instrlib>:"niDCPower Abort With Channels.vi"("error in (no error)"=w316, "channel name"=w300, "instrument handle"=w301) -> ("error out"=w314:errorcluster, "instrument handle out"=w313:refnum<k15>)  [unwired: 7 in]
                n104 = call <instrlib>:"niDCPower Reset With Channels.vi"("error in (no error)"=w314, "channel name"=w300, "instrument handle"=w313) -> ("error out"=w308:errorcluster, "instrument handle out"=w309:refnum<k15>)  [unwired: 7 in]
                n105 = call <instrlib>:"niDCPower Close.vi"("error in (no error)"=w308, "instrument handle"=w309) -> ("error out"=w304:errorcluster)  [unwired: 9 out]
                n106 = Merge Errors(w304, w306) -> (w305:errorcluster)
              }
            }
            n107 = Bundle By Name(cluster=w283, "Measurement Results.Status"=w281) -> (w282:T3)
          }
        }
      }
    }
    frame "Power off the DUT" {
      # "Stops generation on the output channel and resets the channels to default values"
      n108 = Unbundle By Name(w332) -> ("Source resource name"=w353:string, "Load resource name"=w350:string)
      n109 = call <instrlib>:"niDCPower Initialize With Independent Channels.vi"("error in (no error)"=w331, "resource name"=w350) -> ("error out"=w349:errorcluster, "instrument handle out"=w351:refnum<k15>)  [unwired: 8 in]
      n110 = call-poly <instrlib>:"niDCPower Get Channel Name (Poly).vi"("error in (no error)"=w349, "index"="0", "instrument handle"=w351) -> ("error out"=w342:errorcluster, "name"=w344:string, "instrument handle out"=w343:refnum<k15>)  [unwired: 6 in]
      n111 = call <instrlib>:"niDCPower Configure Output Enabled.vi"("error in (no error)"=w342, "output enabled"=FALSE, "channel name"=w344, "instrument handle"=w343) -> ("error out"=w336:errorcluster, "instrument handle out"=w337:refnum<k15>)  [unwired: 6 in]
      n112 = call <instrlib>:"niDCPower Reset With Channels.vi"("error in (no error)"=w336, "channel name"=w344, "instrument handle"=w337) -> ("error out"=w341:errorcluster, "instrument handle out"=w340:refnum<k15>)  [unwired: 7 in]
      n113 = call <instrlib>:"niDCPower Close.vi"("error in (no error)"=w341, "instrument handle"=w340) -> ("error out"=w346:errorcluster)  [unwired: 9 out]
      n114 = call <instrlib>:"niDCPower Initialize With Independent Channels.vi"("error in (no error)"=w346, "resource name"=w353) -> ("error out"=w352:errorcluster, "instrument handle out"=w354:refnum<k15>)  [unwired: 8 in]
      n115 = call-poly <instrlib>:"niDCPower Get Channel Name (Poly).vi"("error in (no error)"=w352, "index"="0", "instrument handle"=w354) -> ("error out"=w347:errorcluster, "name"=w348:string, "instrument handle out"=w345:refnum<k15>)  [unwired: 6 in]
      n116 = call <instrlib>:"niDCPower Reset With Channels.vi"("error in (no error)"=w347, "channel name"=w348, "instrument handle"=w345) -> ("error out"=w338:errorcluster, "instrument handle out"=w339:refnum<k15>)  [unwired: 7 in]
      n117 = call <instrlib>:"niDCPower Close.vi"("error in (no error)"=w338, "instrument handle"=w339) -> ("error out"=w330:errorcluster)  [unwired: 9 out]
      n118 = Bundle By Name(cluster=w329, "Measurement Results.Status"="The DUT is powered OFF" ("message")) -> (w327:T3)
    }
  }
  "error out" <- w8
  "measure call context out" <- w6
  n119 = Unbundle By Name(w5) -> ("Measurement Results"=→"measurement results":T1)
